vi "Test_pgADO.vi"() -> ()   [LabVIEW 2020]
uses:
  <vilib>/Viviota/shared/ORM_ADONet.lvlibp/ADOMapper/ADOMapper.lvclass
  C:/Program Files/National Instruments/LabVIEW 2020/vi.lib/Viviota/shared/ORM.lvlibp/SqlMapper/SqlMapper.lvclass
  DbConnections/PostgresqlConnection/DBC.lvclass
  C:/Program Files/National Instruments/LabVIEW 2020/vi.lib/Viviota/shared/ORM.lvlibp/DbConnection/DbConnection.lvclass
  <vilib>/Viviota/shared/ORM.lvlibp/TypeMap/TypeMap.lvclass
  <vilib>/Viviota/shared/ORM_lib.lvlibp/ObjectRow/ObjectLUT.lvclass
  <vilib>/numeric/Random Number (Range) I64.vi
  <vilib>/numeric/Random Number (Range) DBL.vi
  f3693442-7653-4e44-a421-498bef5f0c13.vi
  <vilib>/numeric/sub_Random U32.vi
  <vilib>/Viviota/shared/ORM.lvlibp/DbConnection/Write SupportTX.vi
  <vilib>/Viviota/shared/ORM.lvlibp/SqlMapper/Write DbConnection.vi
  <vilib>/JDP Science/JSONtext/Variant to JSON Text.vi
  <vilib>/Viviota/shared/ORM_lib.lvlibp/ObjectRow/Write LUT.vi
  <vilib>/Viviota/shared/ORM.lvlibp/TypeMap/Write Table Name.vi
  <vilib>/Viviota/shared/ORM.lvlibp/TypeMap/Write Autokey.vi
  <vilib>/Viviota/shared/ORM_lib.lvlibp/ObjectRow/Read LUT.vi
  <vilib>/JDP Science/JSONtext/LVClass Serializer/JSONtext LVClass Serializer.lvclass
  <vilib>/Analysis/NI_AALBase.lvlib
  <vilib>/Analysis/baseanly.llb/Mean (DBL).vi
panel:
  out "mean 3":dbl format="%0.6f"
  out "mean 2":dbl format="%0.6f"
  out "mean":dbl format="%0.6f"
  out "x-y":dbl[](array[numeric])
  out "Array 2":dbl[](array[numeric])
  out "Array":dbl[](array[numeric])
  out "LUT 2":variant[](array[variant])
  out "LUT":variant[](array[variant])
  out "id":i32[](array[numeric])
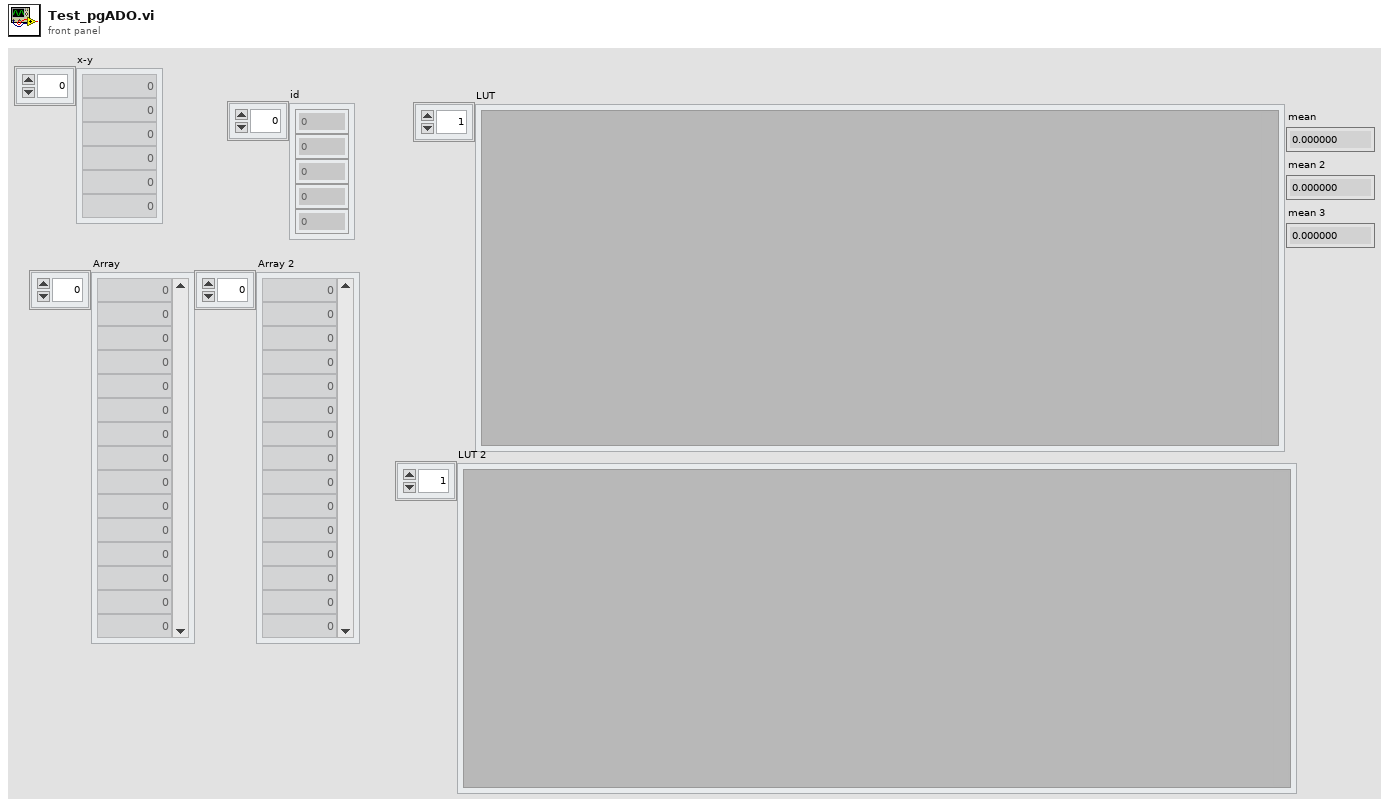
[diagram p1: front panel]
types:
  T1 = cluster{"Text":string, "Integer":i32, "dbl":dbl, "timestamp":timestamp}
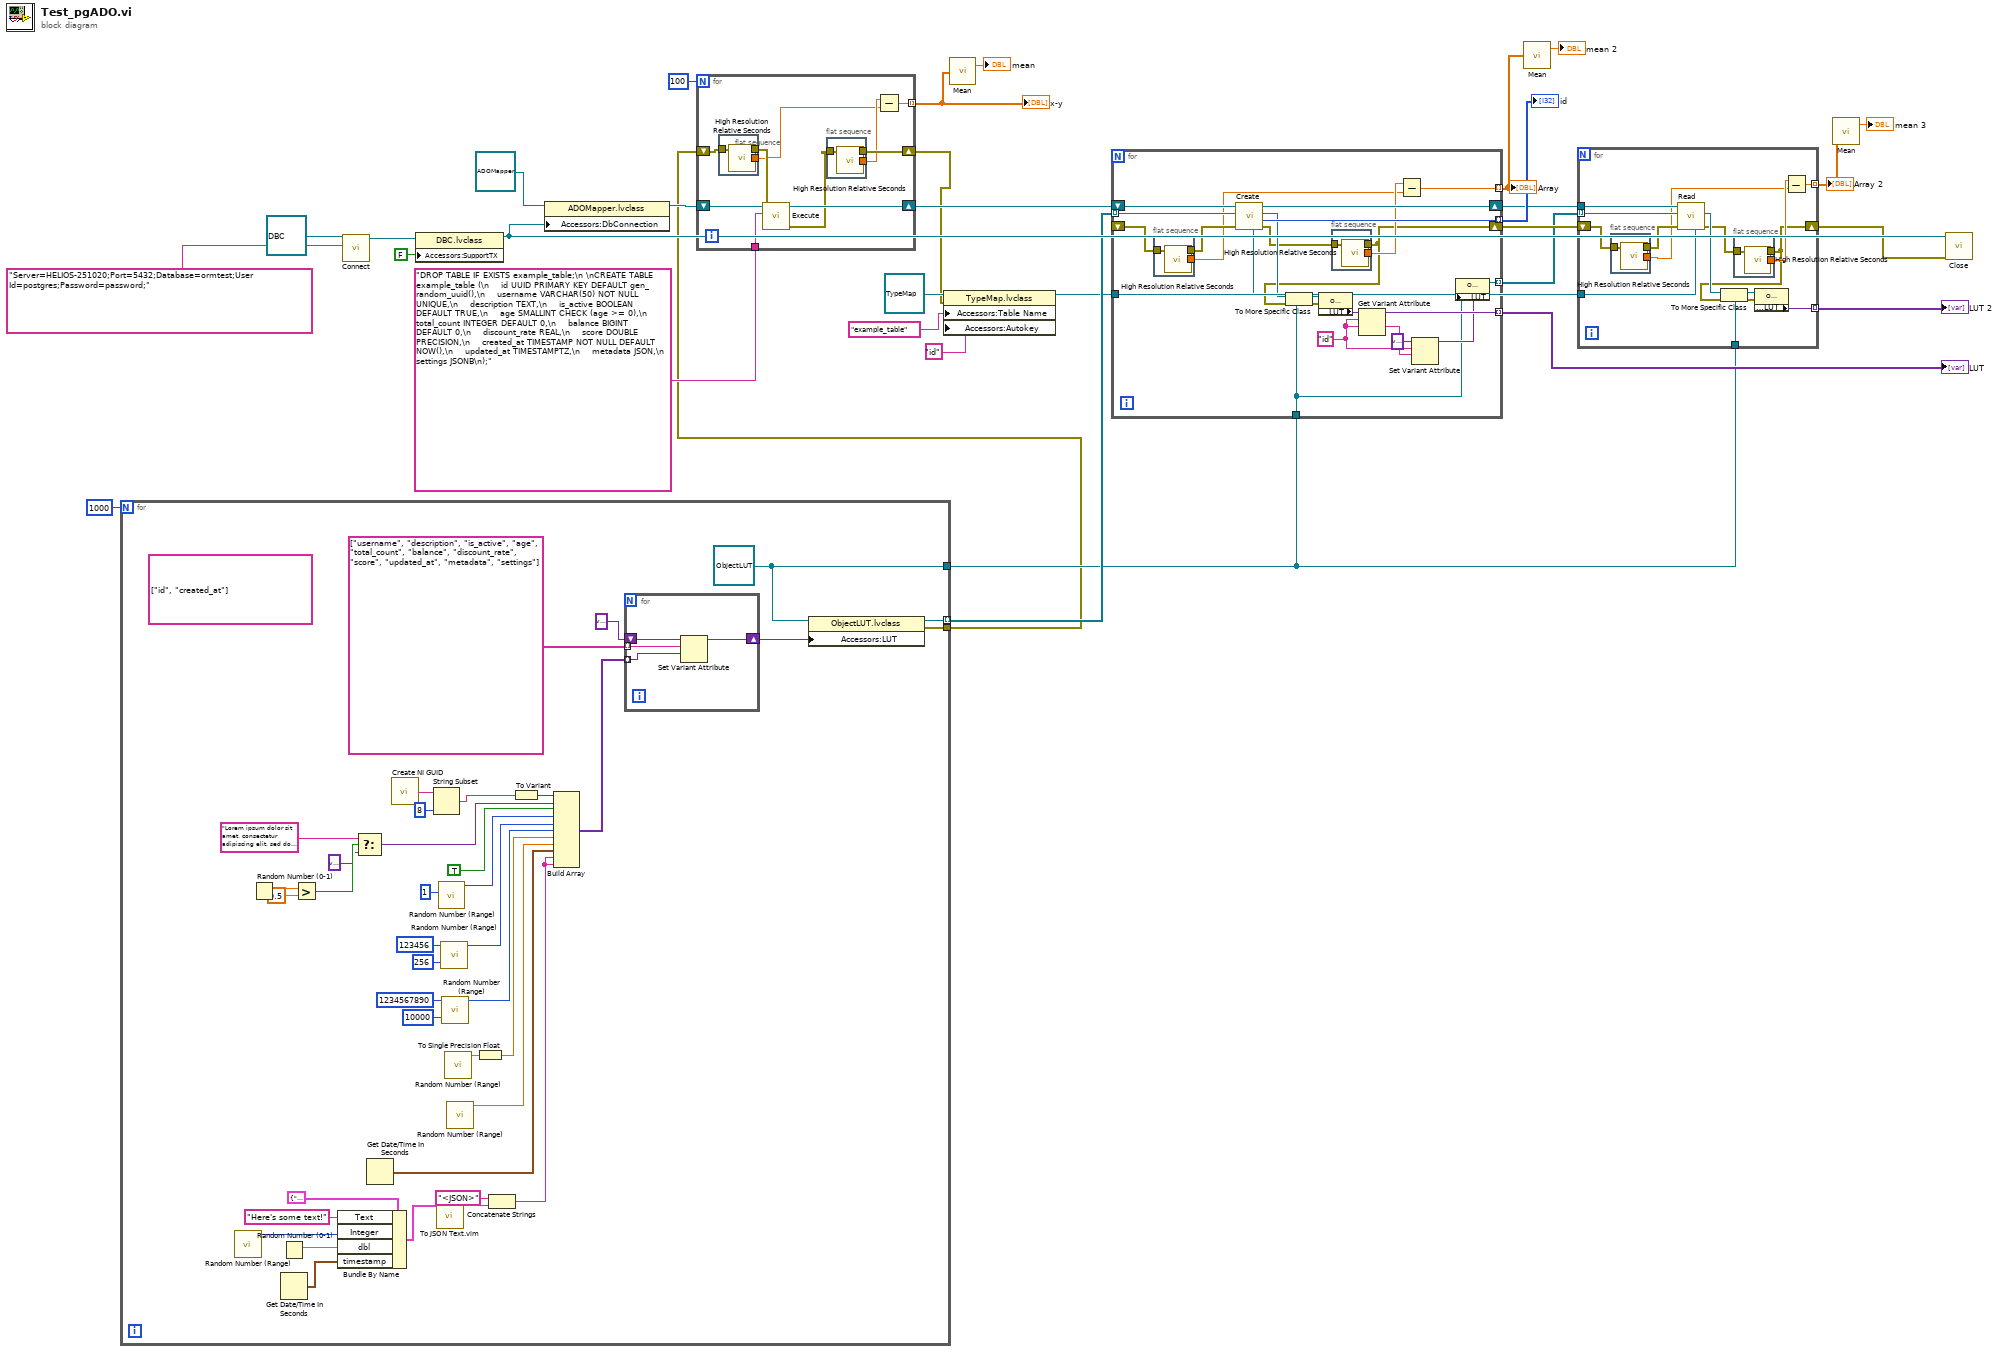
[diagram p0: block diagram]
diagram:
  n1 = for {
    N: 1000 -> [_]
    tunnel: [w39] -> w24 mode=indexing
    tunnel: [w38] -> w14
    tunnel: [w33] -> w9
    w38 = refnum<class "ObjectLUT.lvclass"> refnum ("ORM_lib.lvlibp:ObjectLUT.lvclass")
    (unwired) string[] ["id", "created_at"]
    n2 = call-poly <vilib>:"Random Number (Range).vi"() -> ("number"=w46:i64)  [unwired: 11 in]
    n3 = Random Number (0-1)() -> (number: 0 to 1=w55:dbl)
    n4 = Random Number (0-1)() -> (number: 0 to 1=w47:dbl)
    n5 = Get Date/Time In Seconds() -> (seconds since 1Jan1904=w48:timestamp)
    n6 = Greater?(x=w55, y=0.5) -> (0:w53:bool)
    n7 = Bundle By Name(cluster=T1 {"Text"="This is a test", "Integer"=0, "dbl"=0.0, "timestamp"=timestamp(0 s since 1904-01-01)}, "Text"="Here's some text!", "Integer"=w46, "dbl"=w47, "timestamp"=w48) -> (w44:T1)
    n8 = Select(t="Lorem ipsum dolor sit amet, consectetur adipiscing elit, sed do eiusmod tempor incididunt ut labore et dolore magna aliqua", s=w53, f=variant) -> (s? t:f=w51:variant)
    n9 = Get Date/Time In Seconds() -> (seconds since 1Jan1904=w45:timestamp)
    n10 = call <vilib>:"Create NI GUID.vi"() -> ("NI GUID"=w71:string)
    n11 = String Subset(string=w71, length (rest)=8 ("length (rest)")) -> (substring=w66:string)  [unwired: 1 in]
    n12 = call "To JSON Text.vim"("Anything"=w44) -> ("<JSON>"=w37:string)  [unwired: 9 in, 1 out]
    n13 = call-poly <vilib>:"Random Number (Range).vi"("lower bound (-100)"=i64 1) -> ("number"=w63:i64)  [unwired: 10 in]
    n14 = call-poly <vilib>:"Random Number (Range).vi"("lower bound (-100)"=i64 256, "upper bound (100)"=i64 123456) -> ("number"=w62:i64)  [unwired: 9 in]
    n15 = call-poly <vilib>:"Random Number (Range).vi"("lower bound (-100)"=i64 10000, "upper bound (100)"=i64 1234567890) -> ("number"=w61:i64)  [unwired: 9 in]
    n16 = call-poly <vilib>:"Random Number (Range).vi"() -> ("number"=w59:dbl)  [unwired: 11 in]
    n17 = call-poly <vilib>:"Random Number (Range).vi"() -> ("number"=w57:dbl)  [unwired: 11 in]
    n18 = To Single Precision Float(number=w59) -> (single precision float=w58:sgl)
    n19 = Concatenate Strings("<JSON>" ("string"), w37) -> (w36:string)
    n20 = To Variant(anything=w66) -> (Variant=w65:variant)
    n21 = Build Array(w65, w51, TRUE, w63, w62, w61, w58, w57, w45, w36, w36) -> (w42:variant[])
    n22 = for {
      tunnel: string[] ["username", "description", "is_active", "age", "total_count", "balance", "discount_rate", "score", "updated_at", "metadata", "settings"] -> [w75] mode=indexing
      tunnel: w42 -> [w74] mode=indexing
      shift-right: [w73] -> w40
      shift-left: variant -> [w72]
      n23 = Set Variant Attribute(Variant=w72, name=w75, value=w74) -> (Variant out=w73:variant)  [unwired: 1 in, 2 out]
    }
    n24 = property class="ObjectLUT.lvclass"(reference=w38, "Accessors:LUT"=w40) -> (reference out=w39:refnum<class "ObjectLUT.lvclass">, error out=w33:errorcluster)  [unwired: 1 in]
  }
  n25 = call-dynamic "Connect.vi"("Connection String"="Server=HELIOS-251020;Port=5432;Database=ormtest;User Id=postgres;Password=password;", "PostgresqlConnection in"=refnum<class "DBC.lvclass"> refnum) -> ("PostgresqlConnection out"=w30:refnum<class "DBC.lvclass">)  [unwired: 8 in, 1 out]
  n26 = property class="DBC.lvclass"(reference=w30, "Accessors:SupportTX"=FALSE ("SupportTX")) -> (reference out=w25:refnum<class "DBC.lvclass">)  [unwired: 1 in, 1 out]
  n27 = property class="ADOMapper.lvclass"(reference=refnum<class "ADOMapper.lvclass"> refnum ("ORM_ADONet.lvlibp:ADOMapper.lvclass"), "Accessors:DbConnection"=w25) -> (reference out=w27:refnum<class "ADOMapper.lvclass">)  [unwired: 1 in, 1 out]
  n28 = for {
    N: 100 -> [_]
    tunnel: "DROP TABLE IF EXISTS example_table;\n \nCREATE TABLE example_table (\n    id UUID PRIMARY KEY DEFAULT gen_random_uuid(),\n    username VARCHAR(50) NOT NULL UNIQUE,\n    description TEXT,\n    is_active BOOLEAN DEFAULT TRUE,\n    age SMALLINT CHECK (age >= 0),\n    total_count INTEGER DEFAULT 0,\n    balance BIGINT DEFAULT 0,\n    discount_rate REAL,\n    score DOUBLE PRECISION,\n    created_at TIMESTAMP NOT NULL DEFAULT NOW(),\n    updated_at TIMESTAMPTZ,\n    metadata JSON,\n    settings JSONB\n);" ("sql") -> [w84]
    tunnel: [w76] -> w5 mode=indexing
    shift-right: [w83] -> w16
    shift-left: w27 -> [w85]
    shift-right: [w79] -> w8
    shift-left: w9 -> [w82]
    n29 = flat-sequence {
      tunnel: [w89] -> w77
      tunnel: w82 -> [w88]
      tunnel: [w88] -> w81
      frame #0 {
        n30 = call <vilib>:"High Resolution Relative Seconds.vi"() -> ("relative seconds"=w89:dbl)
      }
    }
    n31 = call-dynamic "Execute.vi"("error in (no error)"=w81, "sql"=w84, "ADOMapper in"=w85) -> ("error out"=w80:errorcluster, "ADOMapper out"=w83:refnum<class "ADOMapper.lvclass">)  [unwired: 6 in, 1 out]
    n32 = flat-sequence {
      tunnel: [w87] -> w78
      tunnel: w80 -> [w86]
      tunnel: [w86] -> w79
      frame #0 {
        n33 = call <vilib>:"High Resolution Relative Seconds.vi"() -> ("relative seconds"=w87:dbl)
      }
    }
    n34 = Subtract(x=w78, y=w77) -> (x-y=w76:dbl)
  }
  "x-y" <- w5
  n35 = property class="TypeMap.lvclass"(reference=refnum<class "TypeMap.lvclass"> refnum ("TypeMap in"), error in=w8, "Accessors:Table Name"="example_table" ("Table Name"), "Accessors:Autokey"="id" ("Autokey")) -> (reference out=w15:refnum<class "TypeMap.lvclass">)  [unwired: 1 out]
  n36 = call-poly <vilib>:"Mean.vi"("X"=w5) -> ("mean"=→"mean":dbl)  [unwired: 1 out]
  n37 = for {
    tunnel: w24 -> [w111] mode=indexing
    tunnel: w15 -> [w110]
    tunnel: [w109] -> w21 mode=indexing
    tunnel: w14 -> [w99]
    tunnel: [w104] -> w20 mode=indexing
    shift-right: [w90] -> w18
    shift-left: _ -> [w97]
    tunnel: [w98] -> w17 mode=indexing
    shift-right: [w94] -> w10
    shift-left: w16 -> [w112]
    tunnel: [w91] -> w2 mode=indexing
    w102 = "id" ("name")
    n38 = flat-sequence {
      tunnel: [w116] -> w92
      tunnel: w97 -> [w115]
      tunnel: [w115] -> w96
      frame #0 {
        n39 = call <vilib>:"High Resolution Relative Seconds.vi"() -> ("relative seconds"=w116:dbl)
      }
    }
    n40 = call-dynamic "Create.vi"("TypeMap in"=w110, "error in (no error)"=w96, "object in"=w111, "SqlMapper in"=w112) -> ("error out"=w95:errorcluster, "id"=w109:i32, "object out"=w108:refnum<class>, "SqlMapper out"=w94:refnum<class "SqlMapper.lvclass">)  [unwired: 4 in]
    n41 = To More Specific Class(target class=w99, reference=w108, error in=w90) -> (specific class reference=w106:refnum<class "ObjectLUT.lvclass">, error out=w107:errorcluster)
    n42 = property class="ObjectLUT.lvclass"(reference=w106, error in=w107) -> ("Accessors:LUT"=w105:variant)  [unwired: 2 out]
    n43 = flat-sequence {
      tunnel: [w114] -> w93
      tunnel: w95 -> [w113]
      tunnel: [w113] -> w90
      frame #0 {
        n44 = call <vilib>:"High Resolution Relative Seconds.vi"() -> ("relative seconds"=w114:dbl)
      }
    }
    n45 = Get Variant Attribute(Variant=w105, name=w102, default value (empty Variant)=w102) -> (duplicate Variant=w104:variant, value=w101:string)  [unwired: 1 in, 2 out]
    n46 = Subtract(x=w93, y=w92) -> (x-y=w91:dbl)
    n47 = Set Variant Attribute(Variant=variant ("variant"), name=w102, value=w101) -> (Variant out=w100:variant)  [unwired: 1 in, 2 out]
    n48 = property class="ObjectLUT.lvclass"(reference=w99, "Accessors:LUT"=w100) -> (reference out=w98:refnum<class "ObjectLUT.lvclass">)  [unwired: 1 in, 1 out]
  }
  "id" <- w21
  "LUT" <- w20
  "Array" <- w2
  n49 = call-poly <vilib>:"Mean.vi"("X"=w2) -> ("mean"=→"mean 2":dbl)  [unwired: 1 out]
  n50 = for {
    tunnel: w17 -> [w131] mode=indexing
    tunnel: w10 -> [w130]
    tunnel: w15 -> [w129]
    tunnel: w14 -> [w125]
    tunnel: [w124] -> w13 mode=indexing
    shift-right: [w117] -> w12
    shift-left: w18 -> [w123]
    tunnel: [w118] -> w1 mode=indexing
    n51 = flat-sequence {
      tunnel: [w135] -> w119
      tunnel: w123 -> [w134]
      tunnel: [w134] -> w122
      frame #0 {
        n52 = call <vilib>:"High Resolution Relative Seconds.vi"() -> ("relative seconds"=w135:dbl)
      }
    }
    n53 = call-dynamic "Read.vi"("TypeMap in"=w129, "error in (no error)"=w122, "object in"=w131, "SqlMapper in"=w130) -> ("error out"=w121:errorcluster, "Value"=w126:refnum<class>)  [unwired: 4 in, 2 out]
    n54 = To More Specific Class(target class=w125, reference=w126, error in=w117) -> (specific class reference=w128:refnum<class "ObjectLUT.lvclass">, error out=w127:errorcluster)
    n55 = flat-sequence {
      tunnel: [w133] -> w120
      tunnel: w121 -> [w132]
      tunnel: [w132] -> w117
      frame #0 {
        n56 = call <vilib>:"High Resolution Relative Seconds.vi"() -> ("relative seconds"=w133:dbl)
      }
    }
    n57 = property class="ObjectLUT.lvclass"(reference=w128, error in=w127) -> ("Accessors:LUT"=w124:variant)  [unwired: 2 out]
    n58 = Subtract(x=w120, y=w119) -> (x-y=w118:dbl)
  }
  "LUT 2" <- w13
  "Array 2" <- w1
  n59 = call-poly <vilib>:"Mean.vi"("X"=w1) -> ("mean"=→"mean 3":dbl)  [unwired: 1 out]
  n60 = call-dynamic "Close.vi"("error in (no error)"=w12, "dbcDotNet in"=w25) -> ()  [unwired: 9 in, 1 out]
